vi "Test Server.vi"() -> ()   [LabVIEW 2020]
uses:
  source/PV Data/NT Base/NT Base.lvclass
  source/Server/Server/Server.lvclass
  <vilib>/numeric/Random Number (Range) I64.vi
  source/Server/Server/Fetch - NT.vi
  source/Server/Server/Add PV - Any Class.vi
  source/Server/Server/Post - Any Class.vi
panel:
  out "Probe":T1
  in  "PV":u16(ring) items=["DEV:BOOL", "DEV:BOOL_ARRAY", "DEV:ENUM", "DEV:FLOAT32", "DEV:FLOAT32_ARRAY", "DEV:FLOAT64", "DEV:FLOAT64_ARRAY", "DEV:INT16", "DEV:INT16_ARRAY", "DEV:INT32", "DEV:INT32_ARRAY", "DEV:INT64", "DEV:INT64_ARRAY", "DEV:INT8", "DEV:INT8_ARRAY", "DEV:STRING", "DEV:STRING_ARRAY", "DEV:UINT16", "DEV:UINT16_ARRAY", "DEV:UINT32", "DEV:UINT32_ARRAY", "DEV:UINT64", "DEV:UINT64_ARRAY", "DEV:UINT8", "DEV:UINT8_ARRAY"]
  in  "Update":bool caption="Update values"
  in  "stop":bool
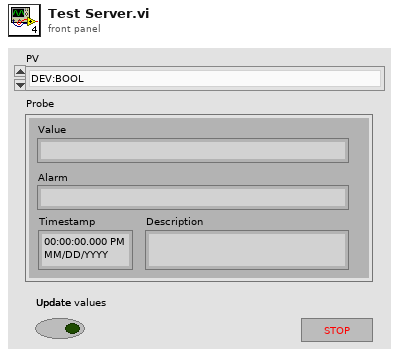
[diagram p1: front panel]
types:
  T1 = cluster{"Timestamp":timestamp, "Value":string, "Description":string, "Alarm":string}
  T2 = typedef "PV Access.lvlib/PV Data.lvlib/Probe.ctl" = cluster{"Timestamp":timestamp, "Value":string, "Description":string, "Alarm":string}
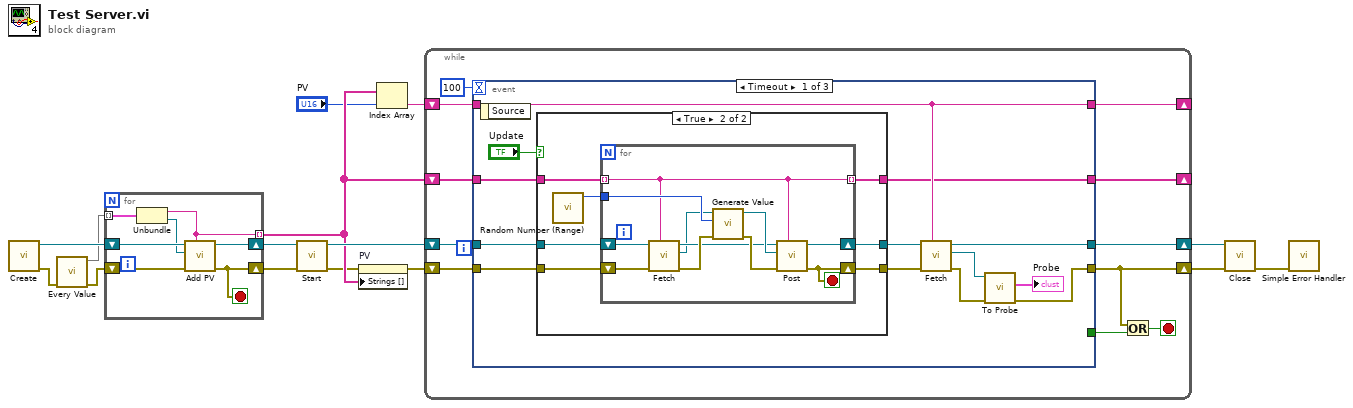
[diagram p0: block diagram]
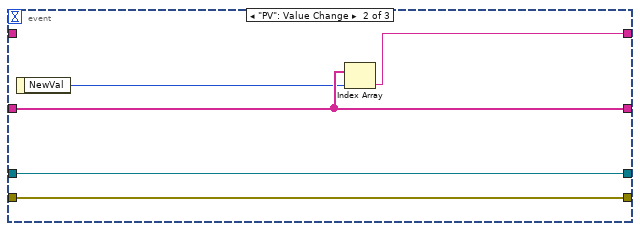
[diagram p3: hidden frame]
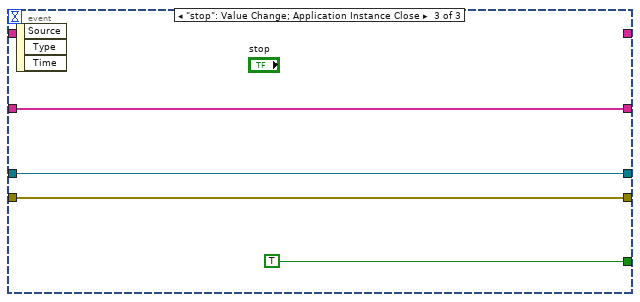
[diagram p4: hidden frame]
diagram:
  n1 = call "Create.vi"() -> ("error out"=w7:errorcluster, "Server out"=w6:refnum<class "Server.lvclass">)  [unwired: 10 in]
  n2 = call "Every Value.vi"("error in (no error)"=w7) -> ("error out"=w5:errorcluster, "values"=w4:map{string, refnum<class "NT Base.lvclass">})  [unwired: 9 in]
  n3 = for {
    shift-right: [w22] -> w14
    shift-left: w6 -> [w20]
    tunnel: [w17] -> w9 mode=indexing
    shift-right: [w21] -> w3
    shift-left: w5 -> [w19]
    tunnel: w4 -> [w18] mode=indexing
    stop <- w21 stop-if-true
    n4 = Unbundle(w18) -> ("PV name"=w17:string, "PV Data.lvlib:NT Base.lvclass"=w16:refnum<class "NT Base.lvclass">)
    n5 = call-poly "Add PV.vi"("PV name"=w17, "error in (no error)"=w19, "initial value"=w16, "Server in"=w20) -> ("error out"=w21:errorcluster, "Server out"=w22:refnum<class "Server.lvclass">)  [unwired: 5 in, 1 out]
  }
  n6 = call-dynamic "Start.vi"("error in (no error)"=w3, "Server in"=w14) -> ("error out"=w2:errorcluster, "Server out"=w15:refnum<class "Server.lvclass">)  [unwired: 8 in]
  n7 = property on="PV" class="Ring (strict)"(error in=w2, "Strings []"=w9) -> (error out=w1:errorcluster)  [unwired: 1 in, 1 out]
  n8 = Index Array(array=w9, index="PV") -> (element=w10:string)
  n9 = while {
    shift-right: [w28] -> w13
    shift-left: w1 -> [w33]
    shift-right: [w31] -> w12
    shift-left: w15 -> [w32]
    shift-right: [w25] -> _
    shift-left: w9 -> [w26]
    shift-right: [w24] -> _
    shift-left: w10 -> [w23]
    stop <- w30 stop-if-true
    n10 = event shown="[0] Timeout" {
      selector: _ -> [_ _ _]
      dyn-events: _ -> [_ _ _]
      timeout: 100 -> [_ _ _]
      tunnel: [w37 w71 w76] -> w28
      tunnel: w33 -> [w45 w71 w76]
      tunnel: w32 -> [w46 w72 w75]
      tunnel: [w35 w72 w75] -> w31
      tunnel: [_ _ TRUE] -> w29
      tunnel: w26 -> [w43 w69 w73]
      tunnel: [w39 w69 w73] -> w25
      tunnel: [w40 w70 _] -> w24
      tunnel: w23 -> [w40 _ _]
      event Timeout {
        n11 = event-data() -> ()  [unwired: 1 in, 1 out]
        n12 = case shown="True" "Update" {
          tunnel: w46 -> [w49 w56]
          tunnel: [w49 w55] -> w41
          tunnel: w45 -> [w48 w54]
          tunnel: [w48 w53] -> w42
          tunnel: w43 -> [w47 w51]
          tunnel: [w47 w50] -> w39
          frame False {
          }
          frame True {
            n13 = call-poly <vilib>:"Random Number (Range).vi"() -> ("number"=w52:i64)  [unwired: 11 in]
            n14 = for {
              shift-right: [w65] -> w53
              shift-left: w54 -> [w62]
              tunnel: w51 -> [w57] mode=indexing
              shift-right: [w67] -> w55
              shift-left: w56 -> [w60]
              tunnel: w52 -> [w66]
              tunnel: [w57] -> w50 mode=indexing
              stop <- w65 stop-if-true
              n15 = call-poly "Fetch.vi"("PV name"=w57, "error in"=w62, "Server in"=w60) -> ("error out"=w61:errorcluster, "value"=w58:refnum<class "NT Base.lvclass">, "Server out"=w59:refnum<class "Server.lvclass">)  [unwired: 5 in, 1 out]
              n16 = call "Generate Value.vi"("error in (no error)"=w61, "base value"=w66, "value in"=w58) -> ("error out"=w63:errorcluster, "value out"=w64:refnum<class "NT Base.lvclass">)  [unwired: 7 in]
              n17 = call-poly "Post.vi"("PV name"=w57, "error in (no error)"=w63, "value in"=w64, "Server in"=w59) -> ("error out"=w65:errorcluster, "Server out"=w67:refnum<class "Server.lvclass">)  [unwired: 5 in, 1 out]
            }
          }
        }
        n18 = call-poly "Fetch.vi"("PV name"=w40, "error in"=w42, "Server in"=w41) -> ("error out"=w38:errorcluster, "value"=w36:refnum<class "NT Base.lvclass">, "Server out"=w35:refnum<class "Server.lvclass">)  [unwired: 5 in, 1 out]
        n19 = call-dynamic "To Probe.vi"("error in (no error)"=w38, "Is Probeable in"=w36) -> ("error out"=w37:errorcluster, "Probe"=→"Probe":T2)  [unwired: 7 in, 1 out]
      }
      event "PV": Value Change {
        n20 = event-data() -> ("NewVal"=w68:u16)  [unwired: 1 in]
        n21 = Index Array(array=w69, index=w68) -> (element=w70:string)
      }
      event "stop": Value Change; Application Instance Close {
        n22 = event-data() -> ()  [unwired: 1 in, 3 out]
      }
    }
    n23 = Or(x=w28, y=w29) -> (x .or. y?=w30:bool)
  }
  n24 = call-dynamic "Close.vi"("error in"=w13, "Server in"=w12) -> ("error out"=w11:errorcluster)  [unwired: 9 in]
  n25 = call <vilib>:"Simple Error Handler.vi"("error in (no error)"=w11) -> ()  [unwired: 4 in, 5 out]
